vi "Export Single VI Help.vi"(6 "Show FP":bool, 8 "error in (no error)":errorcluster, 10 "VI Description":string, 11 "Path":path) -> (0 "error out":errorcluster, 2 "VI Description Out":string)   [LabVIEW 2017, in "csmdoc.lvlib"]
uses:
  csmdoc.lvlib
  _tool/_file/csm-file-support.lvlib
  Communicable State Machine.lvlib
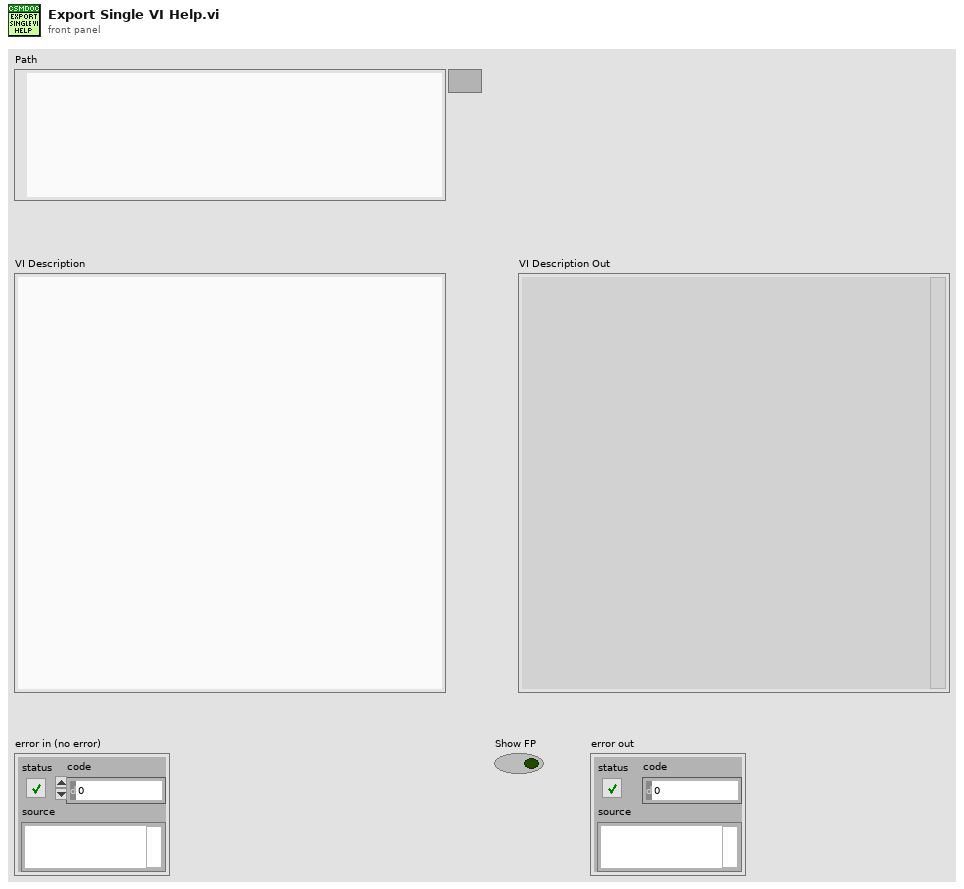
[diagram p1: front panel]
types:
  T1 = typedef "csmdoc.lvlib/DocNote.ctl" = cluster{"ID":string, "Content":string, "Type":string}
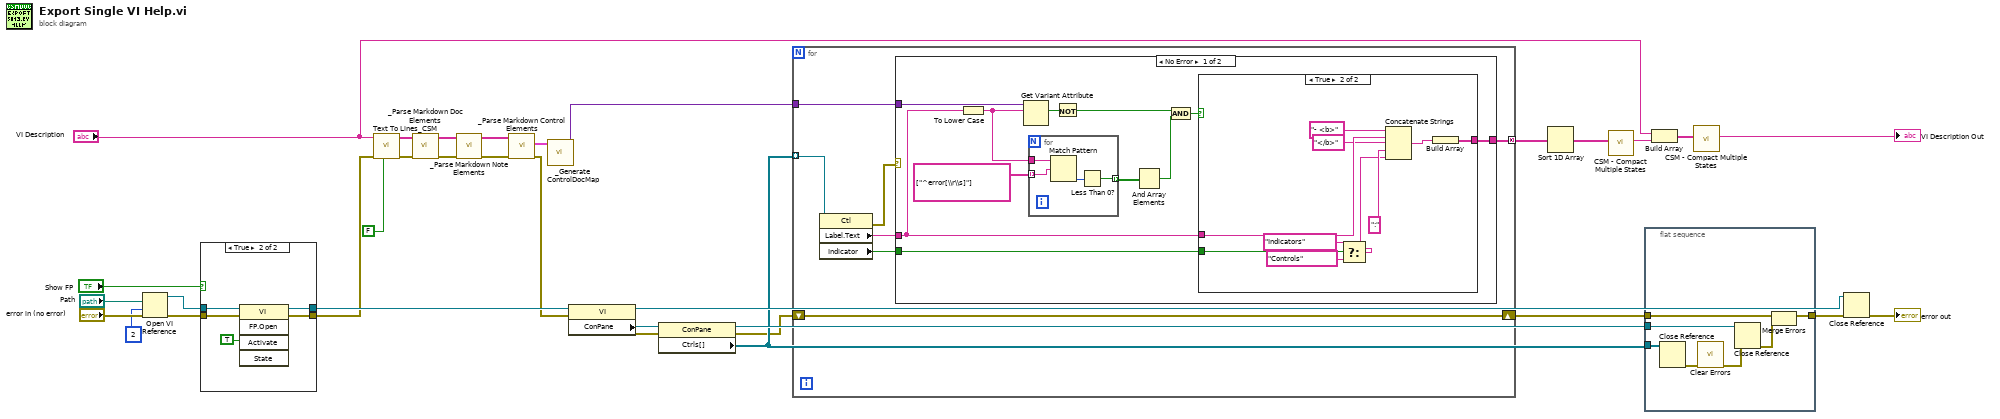
[diagram p0: block diagram]
diagram:
  n1 = Open VI Reference(vi path="Path", options=2, error in (no error)="error in (no error)") -> (vi reference=w27:refnum<vi>, error out=w28:errorcluster)  [unwired: 3 in]
  n2 = case shown="True" "Show FP" {
    tunnel: w28 -> [w34 w39]
    tunnel: w27 -> [w35 w38]
    tunnel: [w34 w37] -> w20
    tunnel: [w35 w36] -> w21
    frame False {
    }
    frame True {
      n3 = invoke class="VI" method="FP.Open"(reference=w38, error in=w39, "Activate"=TRUE ("Activate?")) -> (reference out=w36:refnum<vi>, error out=w37:errorcluster)  [unwired: 2 in, 3 out]
    }
  }
  n4 = call "Text To Lines_CSM.vi"("Remove Empty Lines? (T)"=FALSE ("Remove Empty Lines?(T)"), "error in (no error)"=w20, "String"="VI Description") -> ("error out"=w24:errorcluster, "Lines"=w25:string[])  [unwired: 7 in]
  n5 = call "_Parse Markdown Doc Elements.vi"("Error in"=w24, "Lines"=w25) -> ("Error out"=w22:errorcluster, "Lines (dup)"=w23:string[])  [unwired: 7 in, 1 out]
  n6 = call "_Parse Markdown Note Elements.vi"("Error in"=w22, "Lines"=w23) -> ("Error out"=w3:errorcluster, "Lines (dup)"=w4:string[])  [unwired: 7 in, 1 out]
  n7 = call "_Parse Markdown Control Elements.vi"("Error in"=w3, "Lines"=w4) -> ("Error out"=w2:errorcluster, "Array"=w5:T1[])  [unwired: 7 in, 1 out]
  n8 = call "_Generate ControlDocMap.vi"("Array"=w5) -> ("Variant"=w1:variant)  [unwired: 10 in]
  n9 = property class="VI"(reference=w21, error in=w2) -> (reference out=w16:refnum<vi>, error out=w18:errorcluster, "ConPane"=w19:refnum<vi>)
  n10 = property class="ConPane"(reference=w19, error in=w18) -> (reference out=w17:refnum<vi>, error out=w7:errorcluster, "Ctrls[]"=w14:refnum<vi>[])
  n11 = for {
    tunnel: w1 -> [w46]
    tunnel: w14 -> [w47] mode=indexing
    tunnel: [w43] -> w13 mode=concatenating
    shift-right: [w42] -> w8
    shift-left: w7 -> [w42]
    n12 = property class="Ctl"(reference=w47) -> (error out=w41:errorcluster, "Label.Text"=w45:string, "Indicator"=w44:bool)  [unwired: 1 in, 1 out]
    n13 = case shown="No Error" w41 {
      tunnel: w46 -> [w58 _]
      tunnel: w45 -> [w56 _]
      tunnel: w44 -> [w55 _]
      tunnel: [w54 _] -> w43
      frame No Error {
        n14 = To Lower Case(string=w56) -> (all lower case string=w53:string)
        n15 = Get Variant Attribute(Variant=w58, name=w53) -> (found=w57:bool)  [unwired: 2 in, 3 out]
        n16 = for {
          tunnel: w53 -> [w62]
          tunnel: string[] ["^error[\\r\\s]"] ("string") -> [w61] mode=indexing
          tunnel: [w59] -> w49 mode=indexing
          n17 = Match Pattern(string=w62, regular expression=w61) -> (offset past match=w60:i32)  [unwired: 1 in, 3 out]
          n18 = Less Than 0?(x=w60) -> (x < 0?=w59:bool)
        }
        n19 = Not(x=w57) -> (.not. x?=w51:bool)
        n20 = And Array Elements(Boolean array=w49) -> (logical AND=w48:bool)
        n21 = And(x=w51, y=w48) -> (x .and. y?=w52:bool)
        n22 = case shown="True" w52 {
          tunnel: w56 -> [_ w72]
          tunnel: w55 -> [_ w67]
          tunnel: [_ w68] -> w54
          frame False {
          }
          frame True {
            n23 = Select(t="Indicators" ("string"), s=w67, f="Controls" ("string")) -> (s? t:f=w63:string)
            n24 = Concatenate Strings("- <b>" ("string"), w72, "</b>" ("string"), ":" ("string"), w63) -> (w69:string)
            n25 = Build Array(w69) -> (w68:string[])
          }
        }
      }
      frame Error {
      }
    }
  }
  n26 = Sort 1D Array(array=w13) -> (sorted array=w6:string[])
  n27 = call "CSM - Compact Multiple States.vi"("Multiple States"=w6) -> ("States"=w12:string)  [unwired: 9 in]
  n28 = flat-sequence {
    tunnel: w14 -> [w79]
    tunnel: w17 -> [w78]
    tunnel: [w76] -> w15
    tunnel: w8 -> [w74]
    frame #0 {
      n29 = Close Reference(reference=w79) -> (error out=w77:errorcluster)  [unwired: 1 in]
      n30 = call <vilib>:"Clear Errors.vi"("error in (no error)"=w77) -> ("error out"=w73:errorcluster)  [unwired: 5 in, 1 out]
      n31 = Close Reference(reference=w78, error in (no error)=w73) -> (error out=w75:errorcluster)
      n32 = Merge Errors(w74, w75) -> (w76:errorcluster)
    }
  }
  n33 = Build Array("VI Description", w12) -> (w10:string[])
  n34 = call "CSM - Compact Multiple States.vi"("Multiple States"=w10) -> ("States"=→"VI Description Out":string)  [unwired: 9 in]
  n35 = Close Reference(reference=w16, error in (no error)=w15) -> (error out=→"error out":errorcluster)
